vi "FuncVI_Sub - VI - Recognize LV type descriptor.vi"(6 "error in":errorcluster, 9 "Type Descriptor":i16[](array[numeric]) format="%.0x") -> (0 "error out":errorcluster, 1 "category":enum16{"num", "str"}(ring), 2 "representation":T1(ring), 3 "nDims":i32)   [LabVIEW 2021]
doc: "::: CalcExpress Toolkit :::\nCopyright (c) 2000-2026 Konstantin Shifershteyn. All rights reserved."
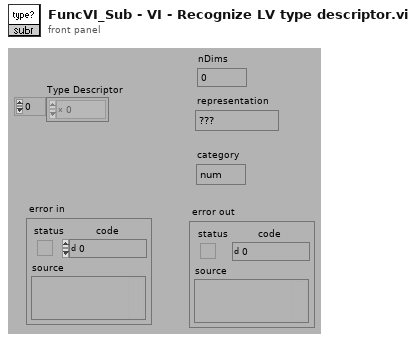
[diagram p1: front panel]
types:
  T1 = enum16{"???", "int8", "int16", "int32", "float32", "float64", "float128", "complex32", "complex64", "complex128", "bool", "string", "path"}
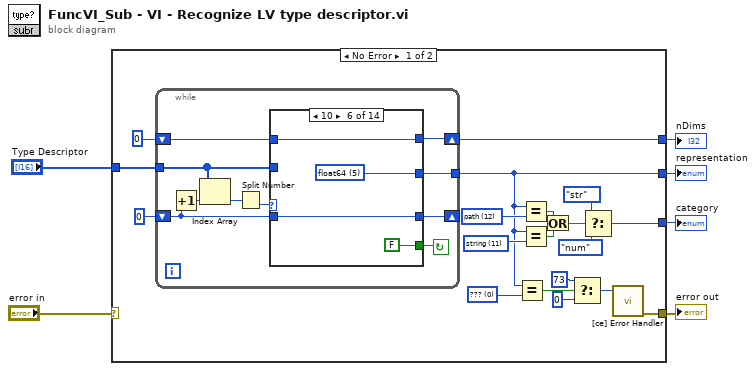
[diagram p0: block diagram]
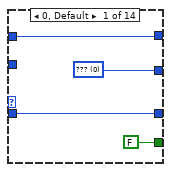
[diagram p2: hidden frame]
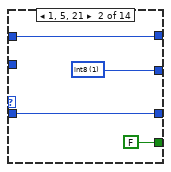
[diagram p3: hidden frame]
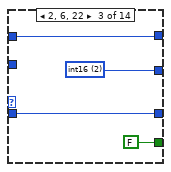
[diagram p4: hidden frame]
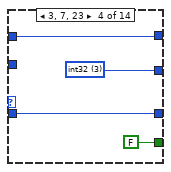
[diagram p5: hidden frame]
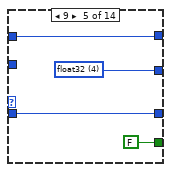
[diagram p6: hidden frame]
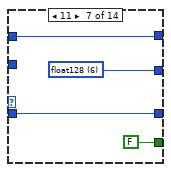
[diagram p7: hidden frame]
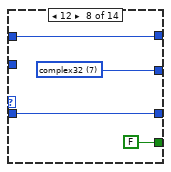
[diagram p8: hidden frame]
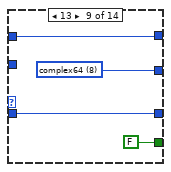
[diagram p9: hidden frame]
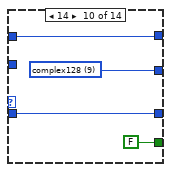
[diagram p10: hidden frame]
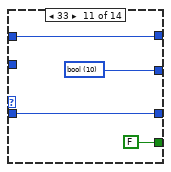
[diagram p11: hidden frame]
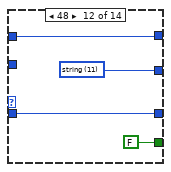
[diagram p12: hidden frame]
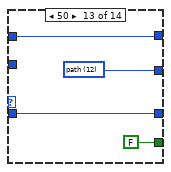
[diagram p13: hidden frame]
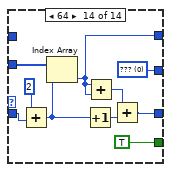
[diagram p14: hidden frame]
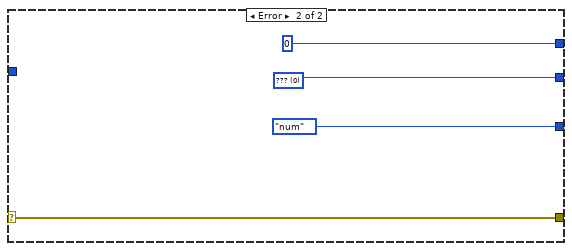
[diagram p15: hidden frame]
diagram:
  n1 = case shown="No Error" "error in" {
    selector: "error in" -> [_ w98]
    tunnel: "Type Descriptor" -> [w23 _]
    tunnel: [w22 0] -> w5
    tunnel: [w16 enum16{"num", "str"}."num" ("category")] -> w4
    tunnel: [w13 w99] -> w3
    tunnel: [w7 w98] -> w2
    frame No Error {
      w21 = u16 12 items=["???", "int8", "int16", "int32", "float32", "float64", "float128", "complex32", "complex64", "complex128", "bool", "string", "path"] ("representation")
      w20 = u16 11 items=["???", "int8", "int16", "int32", "float32", "float64", "float128", "complex32", "complex64", "complex128", "bool", "string", "path"] ("representation")
      w12 = u16 0 items=["???", "int8", "int16", "int32", "float32", "float64", "float128", "complex32", "complex64", "complex128", "bool", "string", "path"] ("representation")
      n2 = while {
        tunnel: [w28] -> w13
        tunnel: w23 -> [w33]
        shift-left: 0 -> [w29]
        shift-right: [w30] -> w22
        shift-left: 0 -> [w32]
        shift-right: [w31] -> _
        stop <- w26 continue-if-true
        n3 = Increment(x=w32) -> (x+1=w27:i32)
        n4 = Index Array(array=w33, index=w27) -> (element=w35:i16)
        n5 = Split Number(x=w35) -> (lo(x)=w34:u8)  [unwired: 1 out]
        n6 = case shown="10" w34 {
          tunnel: w33 -> [_ _ _ _ _ _ _ _ _ _ _ _ _ w97]
          tunnel: w32 -> [w39 w43 w47 w51 w55 w59 w63 w67 w71 w75 w79 w83 w87 w91]
          tunnel: [w39 w43 w47 w51 w55 w59 w63 w67 w71 w75 w79 w83 w87 w95] -> w31
          tunnel: [w38 w42 w46 w50 w54 w58 w62 w66 w70 w74 w78 w82 w86 w96] -> w30
          tunnel: w29 -> [w38 w42 w46 w50 w54 w58 w62 w66 w70 w74 w78 w82 w86 _]
          tunnel: [w37 w41 w45 w49 w53 w57 w61 w65 w69 w73 w77 w81 w85 w92] -> w28
          tunnel: [FALSE FALSE FALSE FALSE FALSE FALSE FALSE FALSE FALSE FALSE FALSE FALSE FALSE TRUE] -> w26
          frame 0, Default {
            w37 = u16 0 items=["???", "int8", "int16", "int32", "float32", "float64", "float128", "complex32", "complex64", "complex128", "bool", "string", "path"] ("representation")
          }
          frame 1, 5, 21 {
            w41 = u16 1 items=["???", "int8", "int16", "int32", "float32", "float64", "float128", "complex32", "complex64", "complex128", "bool", "string", "path"] ("representation")
          }
          frame 2, 6, 22 {
            w45 = u16 2 items=["???", "int8", "int16", "int32", "float32", "float64", "float128", "complex32", "complex64", "complex128", "bool", "string", "path"] ("representation")
          }
          frame 3, 7, 23 {
            w49 = u16 3 items=["???", "int8", "int16", "int32", "float32", "float64", "float128", "complex32", "complex64", "complex128", "bool", "string", "path"] ("representation")
          }
          frame 9 {
            w53 = u16 4 items=["???", "int8", "int16", "int32", "float32", "float64", "float128", "complex32", "complex64", "complex128", "bool", "string", "path"] ("representation")
          }
          frame 10 {
            w57 = u16 5 items=["???", "int8", "int16", "int32", "float32", "float64", "float128", "complex32", "complex64", "complex128", "bool", "string", "path"] ("representation")
          }
          frame 11 {
            w61 = u16 6 items=["???", "int8", "int16", "int32", "float32", "float64", "float128", "complex32", "complex64", "complex128", "bool", "string", "path"] ("representation")
          }
          frame 12 {
            w65 = u16 7 items=["???", "int8", "int16", "int32", "float32", "float64", "float128", "complex32", "complex64", "complex128", "bool", "string", "path"] ("representation")
          }
          frame 13 {
            w69 = u16 8 items=["???", "int8", "int16", "int32", "float32", "float64", "float128", "complex32", "complex64", "complex128", "bool", "string", "path"] ("representation")
          }
          frame 14 {
            w73 = u16 9 items=["???", "int8", "int16", "int32", "float32", "float64", "float128", "complex32", "complex64", "complex128", "bool", "string", "path"] ("representation")
          }
          frame 33 {
            w77 = u16 10 items=["???", "int8", "int16", "int32", "float32", "float64", "float128", "complex32", "complex64", "complex128", "bool", "string", "path"] ("representation")
          }
          frame 48 {
            w81 = u16 11 items=["???", "int8", "int16", "int32", "float32", "float64", "float128", "complex32", "complex64", "complex128", "bool", "string", "path"] ("representation")
          }
          frame 50 {
            w85 = u16 12 items=["???", "int8", "int16", "int32", "float32", "float64", "float128", "complex32", "complex64", "complex128", "bool", "string", "path"] ("representation")
          }
          frame 64 {
            w92 = u16 0 items=["???", "int8", "int16", "int32", "float32", "float64", "float128", "complex32", "complex64", "complex128", "bool", "string", "path"] ("representation")
            n7 = Add(x=2, y=w91) -> (x+y=w89:i32)
            n8 = Index Array(array=w97, index=w89) -> (element=w96:i16)
            n9 = Increment(x=w89) -> (x+1=w93:i32)
            n10 = Add(x=w96, y=w96) -> (x+y=w94:i16)
            n11 = Add(x=w94, y=w93) -> (x+y=w95:i32)
          }
        }
      }
      n12 = Equal?(x=w13, y=w12) -> (x = y?=w11:bool)
      n13 = Equal?(x=w13, y=w21) -> (x = y?=w19:bool)
      n14 = Equal?(x=w13, y=w20) -> (x = y?=w18:bool)
      n15 = Or(x=w19, y=w18) -> (x .or. y?=w17:bool)
      n16 = Select(t=73, s=w11, f=0) -> (s? t:f=w8:i32)
      n17 = Select(t=enum16{"num", "str"}."str" ("category"), s=w17, f=enum16{"num", "str"}."num" ("category")) -> (s? t:f=w16:enum16{"num", "str"})
      n18 = call "[ce] Error Handler.vi"("error code"=w8) -> ("error out"=w7:errorcluster)  [unwired: 9 in, 1 out]
    }
    frame Error {
      w99 = u16 0 items=["???", "int8", "int16", "int32", "float32", "float64", "float128", "complex32", "complex64", "complex128", "bool", "string", "path"] ("representation")
    }
  }
  "nDims" <- w5
  "representation" <- w3
  "category" <- w4
  "error out" <- w2
